vi "Save_Timing_Config.vi"(8 "INI Save Error In":errorcluster caption="错误输入（无错误）", 9 "Save Countdown (s)":dbl=30.0 caption="值", 10 "Save Suspect (s)":dbl=5.0 caption="值", 11 "Save INI File Path":path=path "C:/YOUXI/dazuoye/Config/P1_Runtime.ini" caption="配置文件的路径") -> (3 "INI Save Error":errorcluster caption="错误输出")   [LabVIEW 2020]
uses:
  <vilib>/Utility/config.llb/Open Config Data.vi
  <vilib>/Utility/config.llb/Write Key (Double).vi
  <vilib>/Utility/config.llb/Close Config Data.vi
  <vilib>/Utility/config.llb/NI_LVConfig.lvlib
panel:
  in  "Save Countdown Key":string="CountdownSeconds" caption="键"
  in  "Save Suspect Key":string="SuspectDelaySeconds" caption="键"
  in  "Save INI Section":string="Timing" caption="段"
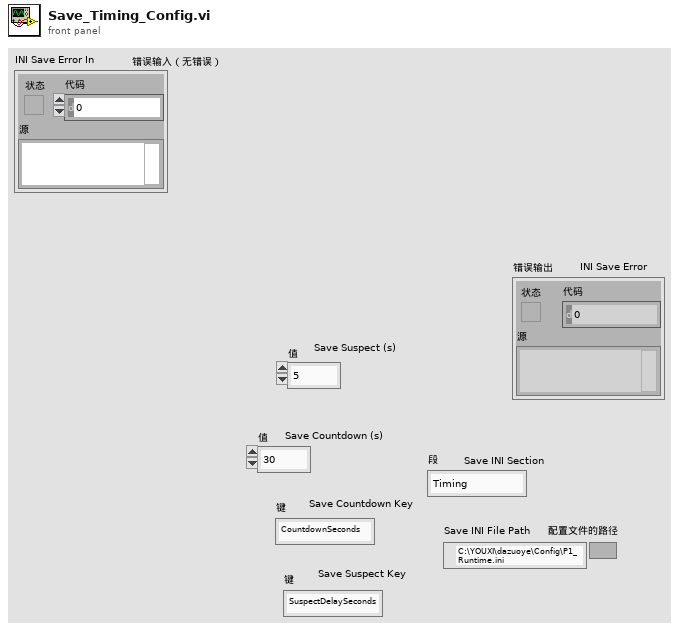
[diagram p1: front panel]
types:
  T1 = typedef "NI_LVConfig.lvlib/Config Data RefNum.ctl" = refnum<k1>
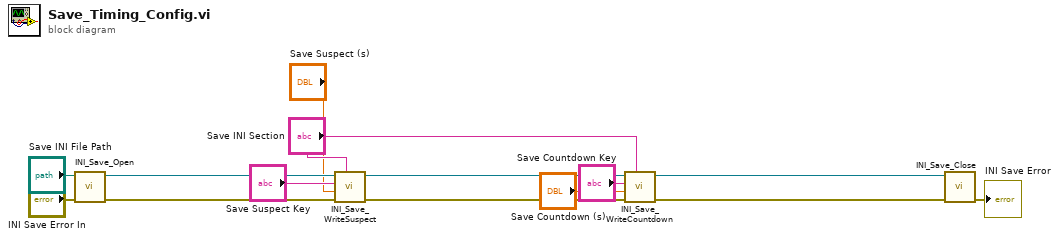
[diagram p0: block diagram]
diagram:
  n1 = call "INI_Save_Open"("error in (no error)"="INI Save Error In", "configuration file path"="Save INI File Path") -> ("error out"=w13:errorcluster, "refnum"=w14:T1)  [unwired: 7 in, 1 out]
  n2 = call "INI_Save_WriteSuspect"("section"="Save INI Section", "error in (no error)"=w13, "value"="Save Suspect (s)", "key"="Save Suspect Key", "refnum"=w14) -> ("error out"=w11:errorcluster, "refnum out"=w12:T1)  [unwired: 4 in, 1 out]
  n3 = call "INI_Save_WriteCountdown"("section"="Save INI Section", "error in (no error)"=w11, "value"="Save Countdown (s)", "key"="Save Countdown Key", "refnum"=w12) -> ("error out"=w9:errorcluster, "refnum out"=w10:T1)  [unwired: 4 in, 1 out]
  n4 = call "INI_Save_Close"("error in (no error)"=w9, "refnum"=w10) -> ("error out"=→"INI Save Error":errorcluster)  [unwired: 8 in, 1 out]
